vi "isNull.vi"(8 "error in (no error)":errorcluster, 11 "NullCustomer in":refnum<class "NullCustomer.lvclass">) -> (0 "error out":errorcluster, 2 "IsNull?":bool, 3 "NullCustomer out":refnum<class "NullCustomer.lvclass">)   [LabVIEW 2018, in "NullCustomer.lvclass"]
uses:
  NullCustomer.lvclass
  AbstractCustomer Class/AbstractCustomer.lvclass
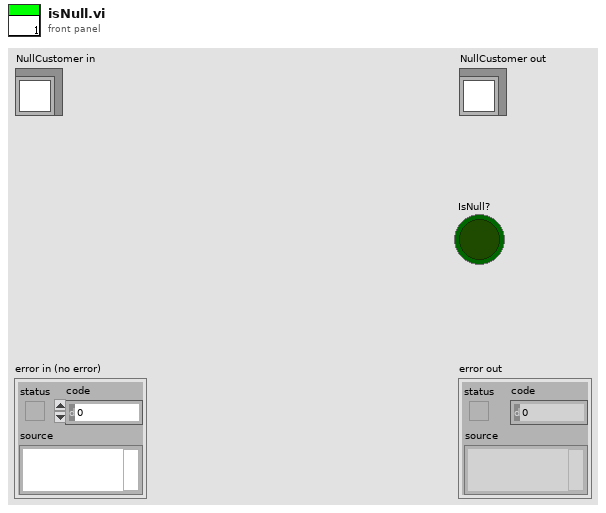
[diagram p1: front panel]
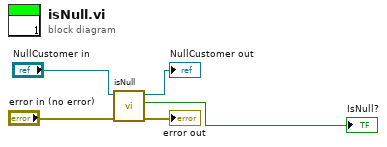
[diagram p0: block diagram]
diagram:
  n1 = call-parent "isNull.vi"("error in (no error)"="error in (no error)", "AbstractCustomer in"="NullCustomer in") -> ("error out"=→"error out":errorcluster, "IsNull?"=→"IsNull?":bool, "AbstractCustomer out"=→"NullCustomer out":refnum<class "NullCustomer.lvclass">)  [unwired: 7 in]
